vi "VIH Utility - STR - String to 1D Str Array.vi"(6 "delimiter ('\\n')":string="\n", 7 "String in":string) -> (3 "Array out":string[](array[string]))   [LabVIEW 2014]
doc: "::: VI Helpeks :::\nCopyright (c) 2000-2026 Konstantin Shifershteyn. All rights reserved."
panel:
  # "VI Helpeks\nCopyright (c) 2012-2026 Konstantin Shifershteyn"
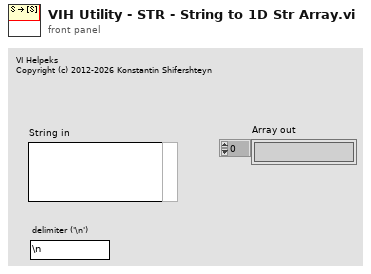
[diagram p1: front panel]
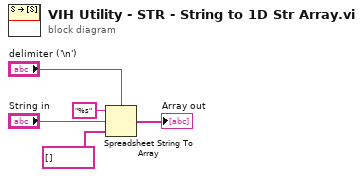
[diagram p0: block diagram]
diagram:
  n1 = Spreadsheet String To Array(delimiter (Tab)="delimiter ('\\n')", format string="%s", spreadsheet string="String in", array type (2D Dbl)=string[] [] ("Array out")) -> (array=→"Array out":string[])
